vi "Check If Pixels Belong In Sector.vi"() -> (3 "FIFO Timeout?":bool)   [LabVIEW 2013]
uses:
  Single Sector Pixel Cluster.ctl
  Globals/Sector Parameter Global.vi
  Globals/Pixel Location Global.vi
  <vilib>/rvi/FIFO/Fifo_Resource/nirvififoEmulationReadFpgaImpl.vi
  <vilib>/rvi/DataTransferAndStorage/Container/Common/niFpgaContainerGetUniqueNameForEmu.vi
  <vilib>/rvi/FIFO/Fifo_Resource/nirvififoEmulationWriteFpgaImpl.vi
  <vilib>/rvi/DataTransferAndStorage/Container/XNode/niFpgaContainer.xnode
  <vilib>/rvi/FIFO/Fifo_Resource/nirvififoEmulationRead.vi
  <vilib>/rvi/FIFO/Fifo_Resource/nirvififoEmulationWrite.vi
  FPGA Image Processing.lvlib
panel:
  out "End of  Data?":bool
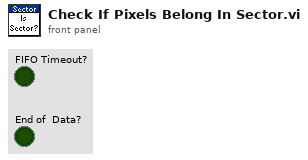
[diagram p1: front panel]
types:
  T1 = typedef "Sector Parameter Cluster.ctl" = cluster{"Start Angle":fxp<+/-,17,2>, "End Angle":fxp<+,17,3>, "Inner Radius":u16, "Outter Radius":u16, "Hinge X":u16, "Hinge Y":u16, "NumWingSectors":u8}
  T2 = typedef "Single Sector Pixel Cluster.ctl" = cluster{"Sector #":u8, "Pixel Value":u8}
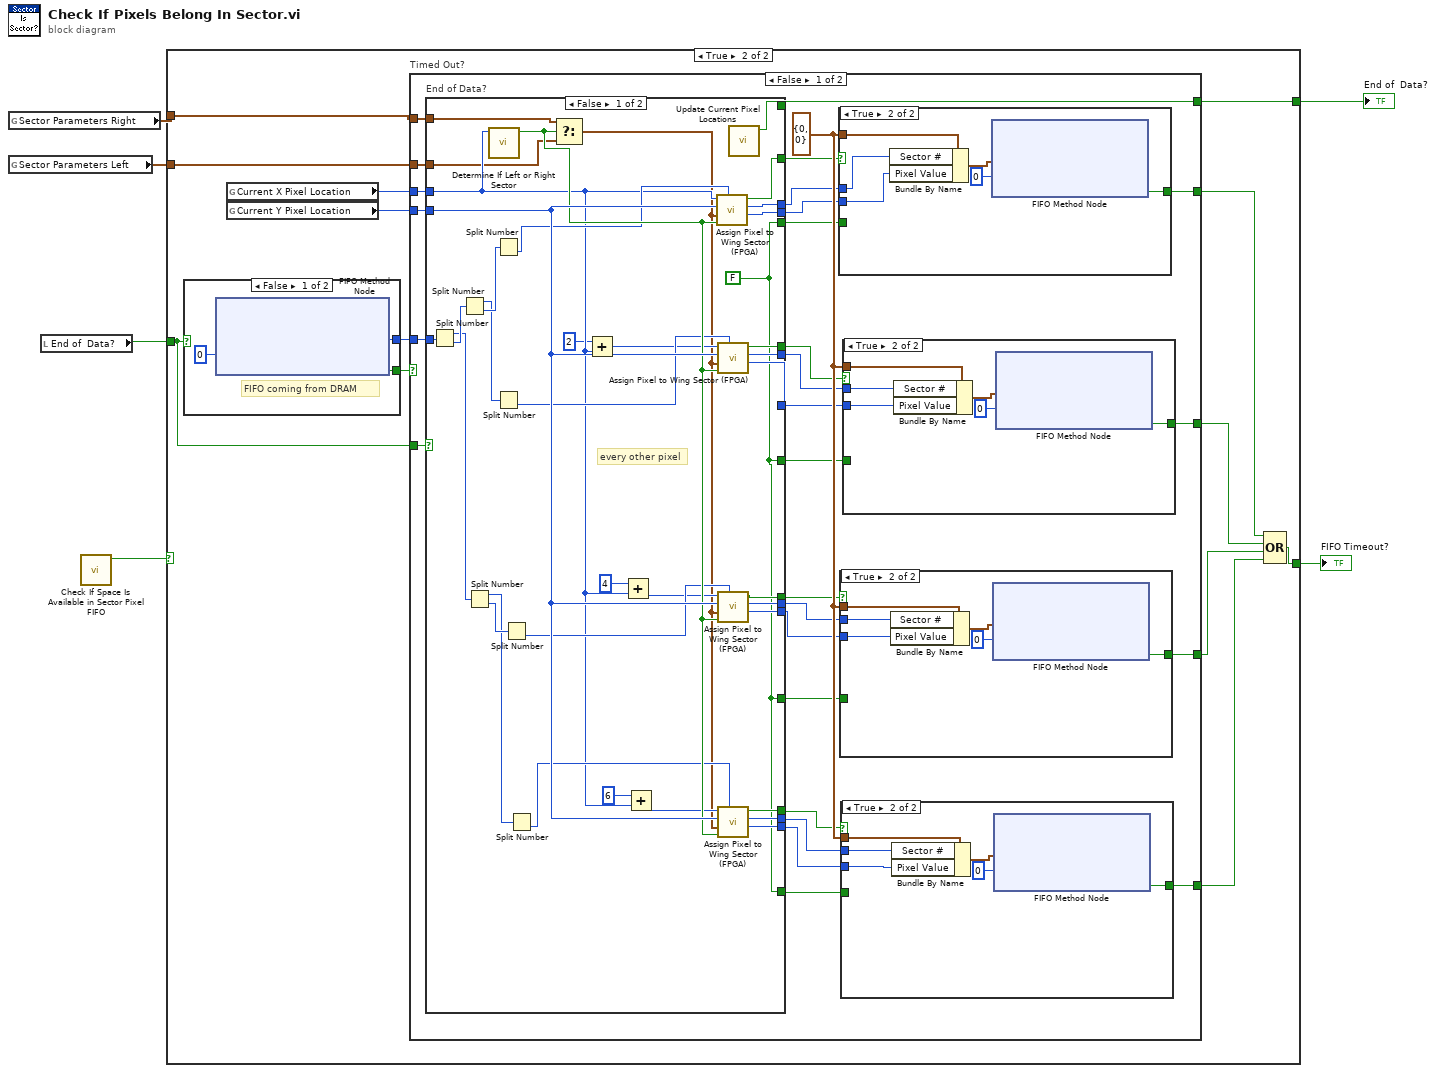
[diagram p0: block diagram]
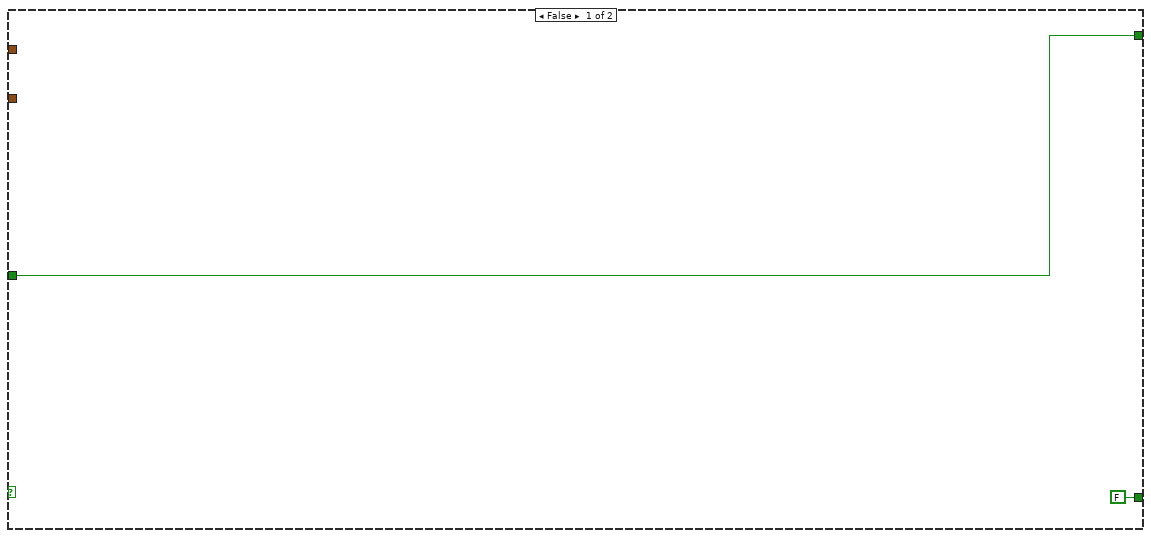
[diagram p2: hidden frame]
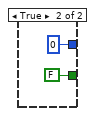
[diagram p3: hidden frame]
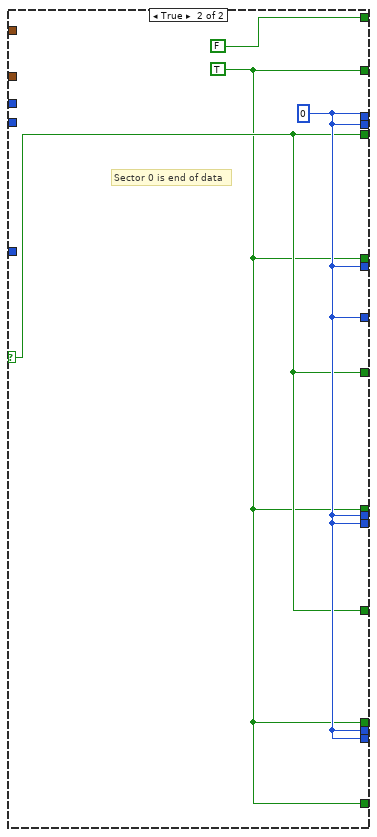
[diagram p4: hidden frame]
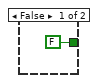
[diagram p5: hidden frame]
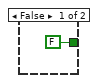
[diagram p6: hidden frame]
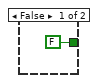
[diagram p7: hidden frame]
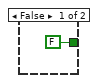
[diagram p8: hidden frame]
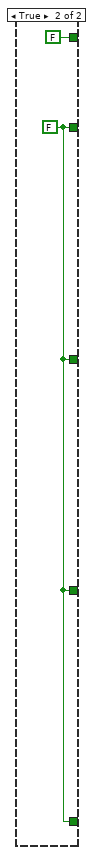
[diagram p9: hidden frame]
diagram:
  n1 = global read "Sector Parameter Global.vi" "Sector Parameters Right"() -> (w2:T1)
  n2 = global read "Sector Parameter Global.vi" "Sector Parameters Left"() -> (w1:T1)
  n3 = local read "End of  Data?"() -> (w4:bool)
  n4 = call "Check If Space Is Available in Sector Pixel FIFO.vi"() -> ("Space Avaliable?"=w3:bool)  [unwired: 11 in]
  n5 = case shown="True" w3 {
    tunnel: [FALSE w13] -> w5
    tunnel: [w8 w12] -> w6
    tunnel: w4 -> [w8 w11]
    tunnel: w2 -> [_ w10]
    tunnel: w1 -> [_ w9]
    frame False {
    }
    frame True {
      n6 = case shown="False" w11 {
        tunnel: [w23 FALSE ("Timed Out?")] -> w21
        tunnel: [w22 u64 0 ("Element")] -> w18
        frame False {
          # "FIFO coming from DRAM"
          n7 = xnode ("FIFO Method Node")("Timeout"=0) -> ("Element"=w22:u64, "Timed Out?"=w23:bool)  [unwired: 1 in, 1 out]
        }
        frame True {
        }
      }
      n8 = global read "Pixel Location Global.vi" "Current X Pixel Location"() -> (w20:u16)
      n9 = global read "Pixel Location Global.vi" "Current Y Pixel Location"() -> (w19:u16)
      n10 = case "Timed Out?" shown="False" w21 {
        tunnel: w20 -> [w45 _]
        tunnel: w19 -> [w54 _]
        tunnel: w18 -> [w52 _]
        tunnel: [w53 w125] -> w17
        tunnel: [w51 w125] -> w16
        tunnel: [w50 w125] -> w15
        tunnel: [w48 w125] -> w14
        tunnel: w10 -> [w47 _]
        tunnel: w9 -> [w46 _]
        tunnel: [w32 FALSE ("End of Average Data?")] -> w12
        tunnel: w11 -> [w31 _]
        frame False {
          w49 = T2 {"Sector #"=0, "Pixel Value"=0} ("Single Sector Pixel")
          n11 = case "End of Data?" shown="False" w31 {
            selector: w31 -> [_ w93]
            tunnel: w54 -> [w91 _]
            tunnel: w52 -> [w87 _]
            tunnel: w47 -> [w57 _]
            tunnel: w46 -> [w56 _]
            tunnel: w45 -> [w65 _]
            tunnel: [w81 w92] -> w44
            tunnel: [w80 w94] -> w43
            tunnel: [w79 w94] -> w42
            tunnel: [w78 w92] -> w41
            tunnel: [w77 w94] -> w40
            tunnel: [w75 w94] -> w39
            tunnel: [w74 w92] -> w38
            tunnel: [w73 w94] -> w37
            tunnel: [w71 w94] -> w36
            tunnel: [w70 w92] -> w35
            tunnel: [w69 w94] -> w34
            tunnel: [w68 w94] -> w33
            tunnel: [w66 FALSE ("End of data?")] -> w32
            tunnel: [w64 w93] -> w30
            tunnel: [w64 w93] -> w29
            tunnel: [w64 w93] -> w28
            tunnel: [w64 w92] -> w27
            frame False {
              w64 = FALSE
              # "every other pixel"
              n12 = Split Number(x=w87) -> (hi(x)=w89:u32, lo(x)=w90:u32)
              n13 = Split Number(x=w90) -> (hi(x)=w86:u16, lo(x)=w88:u16)
              n14 = Split Number(x=w89) -> (hi(x)=w84:u16, lo(x)=w85:u16)
              n15 = call "Determine If Left or Right Sector.vi"("X Pixel Location"=w65) -> ("Right Sector?"=w83:bool)  [unwired: 10 in]
              n16 = Split Number(x=w88) -> (lo(x)=w82:u8)  [unwired: 1 out]
              n17 = Split Number(x=w86) -> (lo(x)=w76:u8)  [unwired: 1 out]
              n18 = Split Number(x=w85) -> (lo(x)=w72:u8)  [unwired: 1 out]
              n19 = Split Number(x=w84) -> (lo(x)=w67:u8)  [unwired: 1 out]
              n20 = Select(t=w57, s=w83, f=w56) -> (s? t:f=w55:T1)
              n21 = Add(x=u16 2, y=w65) -> (x+y=w60:u16)
              n22 = Add(x=u16 4, y=w65) -> (x+y=w59:u16)
              n23 = Add(x=u16 6, y=w65) -> (x+y=w58:u16)
              n24 = call "Assign Pixel to Wing Sector (FPGA).vi"("Pixel Intensity In"=w82, "Right Wing?"=w83, "Sector Parameters"=w55, "Pixel Y"=w91, "Pixel X"=w65) -> ("Pixel Intensity Out"=w79:u8, "sector #"=w80:u8, "output valid"=w81:bool)  [unwired: 3 in]
              n25 = call "Assign Pixel to Wing Sector (FPGA).vi"("Pixel Intensity In"=w76, "Right Wing?"=w83, "Sector Parameters"=w55, "Pixel Y"=w91, "Pixel X"=w60) -> ("Pixel Intensity Out"=w75:u8, "sector #"=w77:u8, "output valid"=w78:bool)  [unwired: 3 in]
              n26 = call "Assign Pixel to Wing Sector (FPGA).vi"("Pixel Intensity In"=w72, "Right Wing?"=w83, "Sector Parameters"=w55, "Pixel Y"=w91, "Pixel X"=w59) -> ("Pixel Intensity Out"=w71:u8, "sector #"=w73:u8, "output valid"=w74:bool)  [unwired: 3 in]
              n27 = call "Assign Pixel to Wing Sector (FPGA).vi"("Pixel Intensity In"=w67, "Right Wing?"=w83, "Sector Parameters"=w55, "Pixel Y"=w91, "Pixel X"=w58) -> ("Pixel Intensity Out"=w68:u8, "sector #"=w69:u8, "output valid"=w70:bool)  [unwired: 3 in]
              n28 = call "Update Current Pixel Locations.vi"() -> ("End of data?"=w66:bool)  [unwired: 11 in]
            }
            frame True {
              w94 = u8 0 ("sector #")
              w92 = TRUE ("output valid")
              # "Sector 0 is end of data"
            }
          }
          n29 = case shown="True" w44 {
            tunnel: w49 -> [_ w118]
            tunnel: [FALSE ("Timed Out?") w121] -> w53
            tunnel: w43 -> [_ w119]
            tunnel: w42 -> [_ w120]
            tunnel: w30 -> [_ _]
            frame False {
            }
            frame True {
              n30 = Bundle By Name(cluster=w118, "Sector #"=w119, "Pixel Value"=w120) -> (w122:T2)
              n31 = xnode ("FIFO Method Node")("Element"=w122, "Timeout"=0) -> ("Timed Out?"=w121:bool)  [unwired: 1 in, 1 out]
            }
          }
          n32 = case shown="True" w38 {
            tunnel: w49 -> [_ w109]
            tunnel: [FALSE ("Timed Out?") w106] -> w50
            tunnel: w37 -> [_ w104]
            tunnel: w36 -> [_ w105]
            tunnel: w28 -> [_ _]
            frame False {
            }
            frame True {
              n33 = Bundle By Name(cluster=w109, "Sector #"=w104, "Pixel Value"=w105) -> (w107:T2)
              n34 = xnode ("FIFO Method Node")("Element"=w107, "Timeout"=0) -> ("Timed Out?"=w106:bool)  [unwired: 1 in, 1 out]
            }
          }
          n35 = case shown="True" w35 {
            tunnel: w49 -> [_ w102]
            tunnel: [FALSE ("Timed Out?") w99] -> w48
            tunnel: w34 -> [_ w97]
            tunnel: w33 -> [_ w98]
            tunnel: w27 -> [_ _]
            frame False {
            }
            frame True {
              n36 = Bundle By Name(cluster=w102, "Sector #"=w97, "Pixel Value"=w98) -> (w100:T2)
              n37 = xnode ("FIFO Method Node")("Element"=w100, "Timeout"=0) -> ("Timed Out?"=w99:bool)  [unwired: 1 in, 1 out]
            }
          }
          n38 = case shown="True" w41 {
            tunnel: w49 -> [_ w116]
            tunnel: [FALSE ("Timed Out?") w113] -> w51
            tunnel: w40 -> [_ w111]
            tunnel: w39 -> [_ w112]
            tunnel: w29 -> [_ _]
            frame False {
            }
            frame True {
              n39 = Bundle By Name(cluster=w116, "Sector #"=w111, "Pixel Value"=w112) -> (w114:T2)
              n40 = xnode ("FIFO Method Node")("Element"=w114, "Timeout"=0) -> ("Timed Out?"=w113:bool)  [unwired: 1 in, 1 out]
            }
          }
        }
        frame True {
          w125 = FALSE ("Timed Out?")
        }
      }
      n41 = Compound Arithmetic op=OR(w17, w16, w15, w14) -> (w13:bool)
    }
  }
  "End of  Data?" <- w6
  "FIFO Timeout?" <- w5
